vi "Update Plot Color.vi"(8 "error in (no error)":errorcluster caption="错误输入（无错误）", 11 "Data Viewer 输入":refnum<class "Data Viewer.lvclass">) -> (0 "error out":errorcluster caption="错误输出", 3 "Data Viewer 输出":refnum<class "Data Viewer.lvclass">)   [LabVIEW 2020, in "Data Viewer.lvlib" / "Data Viewer.lvclass"]
uses:
  Data Viewer.lvclass
  Data Viewer.lvclass/Data Viewer.ctl
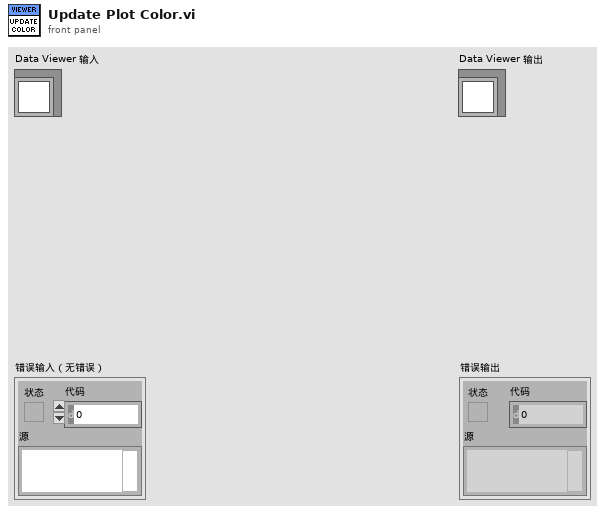
[diagram p1: front panel]
types:
  T1 = typedef "DataSave.lvlib/Data Viewer.lvlib/Data Viewer.lvclass/Legend.ctl" = cluster{"颜色":u32, "曲线名称":string}[]
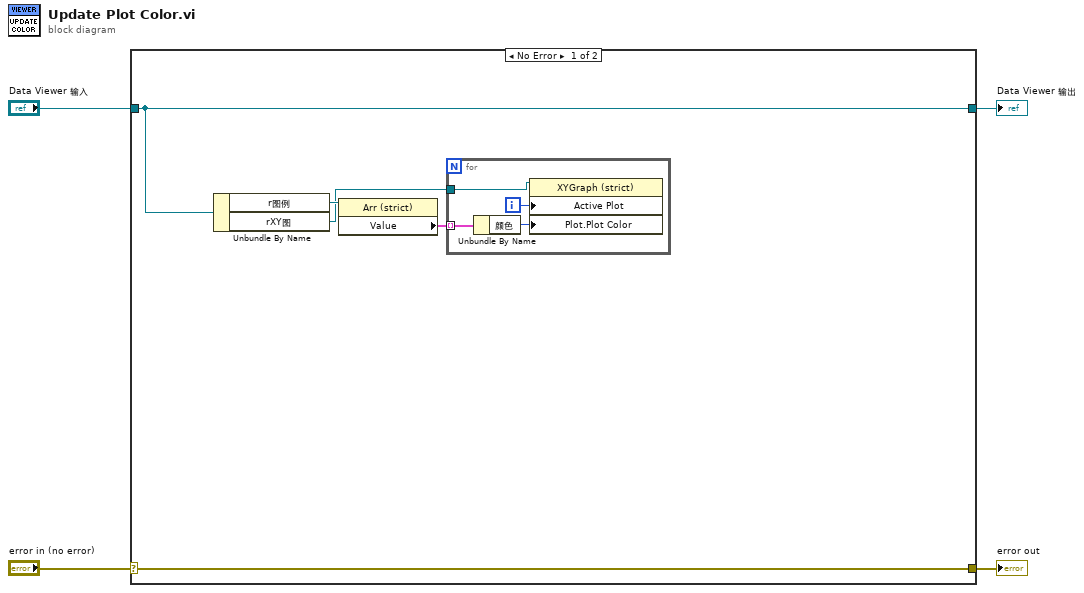
[diagram p0: block diagram]
diagram:
  n1 = case shown="No Error" "error in (no error)" {
    selector: "error in (no error)" -> [w9 w15]
    tunnel: [w9 w15] -> w3
    tunnel: [w8 w14] -> w1
    tunnel: "Data Viewer 输入" -> [w8 w14]
    frame No Error {
      n2 = Unbundle By Name(w8) -> ("r图例"=w7:refnum<vi>, "rXY图"=w5:refnum<vi>)
      n3 = property class="Arr (strict)"(reference=w7) -> ("Value"=w6:T1)  [unwired: 1 in, 2 out]
      n4 = for {
        tunnel: w6 -> [w13] mode=indexing
        tunnel: w5 -> [w12]
        i -> [w10]
        n5 = Unbundle By Name(w13) -> ("颜色"=w11:u32)
        n6 = property class="XYGraph (strict)"(reference=w12, "Active Plot"=w10, "Plot.Plot Color"=w11) -> ()  [unwired: 1 in, 2 out]
      }
    }
    frame Error {
    }
  }
  "error out" <- w3
  "Data Viewer 输出" <- w1
